vi "Conv1D_LabVIEW.vi"(6 "Kernel Relative Size":sgl=0.001, 7 "No. of Repetition":i32, 11 "Size":i32) -> (3 "Results(s)":dbl format="%.6f")   [LabVIEW 2020]
uses:
  4e24d26d-fcbb-44a5-9aa8-75639d06e416.vi
  2ed5783d-9886-4979-abaf-b24675aa47c9.vi
  <vilib>/Utility/High Resolution Relative Seconds.vi
  <vilib>/Analysis/2dsp.llb/1D Convolution (DBL).vi
  <vilib>/Analysis/NI_AALBase.lvlib
  <vilib>/Analysis/NI_AALPro.lvlib
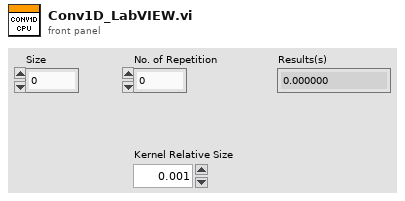
[diagram p1: front panel]
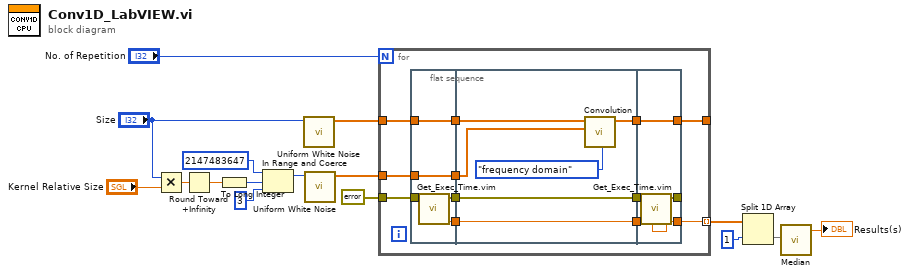
[diagram p0: block diagram]
diagram:
  n1 = Multiply(x="Size", y="Kernel Relative Size") -> (x*y=w12:sgl)
  n2 = Round Toward +Infinity(x=w12) -> (ceil(x): smallest int >= x=w11:sgl)
  n3 = To Long Integer(number=w11) -> (32bit integer=w10:i32)
  n4 = In Range and Coerce(upper limit=2147483647 ("lower limit"), x=w10, lower limit=3) -> (coerced(x)=w14:i32)  [unwired: 1 out]
  n5 = call <vilib>:"Uniform White Noise.vi"("samples"="Size") -> ("uniform white noise"=w5:dbl[])  [unwired: 9 in, 1 out]
  n6 = call <vilib>:"Uniform White Noise.vi"("samples"=w14) -> ("uniform white noise"=w7:dbl[])  [unwired: 9 in, 1 out]
  n7 = for {
    N: "No. of Repetition" -> [_]
    tunnel: w5 -> [w28]
    tunnel: errorcluster {"status"=FALSE, "code"=0, "source"=""} ("error out") -> [w27]
    tunnel: [w20] -> w6 mode=indexing
    tunnel: w7 -> [w19]
    tunnel: [w17] -> _
    n8 = flat-sequence {
      tunnel: w27 -> [w32]
      tunnel: w28 -> [w33]
      tunnel: [w33] -> w26
      tunnel: [w31] -> w25
      tunnel: [w30] -> w21
      tunnel: w19 -> [w29]
      tunnel: [w29] -> w18
      tunnel: w26 -> [w39]
      tunnel: w25 -> [w37]
      tunnel: [w38] -> w24
      tunnel: [w37] -> w23
      tunnel: [w36] -> w22
      tunnel: w21 -> [w36]
      tunnel: w18 -> [w35]
      tunnel: [w42] -> _
      tunnel: [w44] -> w17
      tunnel: w24 -> [w44]
      tunnel: w23 -> [w43]
      tunnel: w22 -> [w41]
      tunnel: [w40] -> w20
      frame #0 {
        n9 = call "Get_Exec_Time.vim"("error in (no error)"=w32) -> ("T(n)"=w30:dbl, "error out"=w31:errorcluster)  [unwired: 6 in, 1 out]
      }
      frame #1 {
        n10 = call-poly <vilib>:"Convolution.vi"("algorithm"=enum32{"direct", "frequency domain"}."frequency domain", "Y"=w35, "X"=w39) -> ("X * Y"=w38:dbl[])  [unwired: 7 in, 1 out]
      }
      frame #2 {
        n11 = call "Get_Exec_Time.vim"("T(n-1)"=w41, "error in (no error)"=w43) -> ("error out"=w42:errorcluster, "dT"=w40:dbl)  [unwired: 5 in, 1 out]
      }
    }
  }
  n12 = Split 1D Array(array=w6, index=1) -> (second subarray=w1:dbl[])  [unwired: 1 out]
  n13 = call <vilib>:"Median.vi"("X"=w1) -> ("median"=→"Results(s)":dbl)  [unwired: 1 out]
